vi "创建任务.vi"(0 "输入通道":tag="Dev2/ai0", 1 "最小测量范围":dbl=-500.0 format="%#_13g", 2 "最大测量范围":dbl=500.0 format="%#_13g", 9 "速率":dbl=200000.0 format="%#_13g", 11 "采样数":i32=2000, 12 "最小输入值":dbl=-2.0 format="%#_13g", 13 "最大输入值":dbl=2.0 format="%#_13g") -> (4 "task out":refnum<k21> caption="任务输出", 6 "采样数out":i32=2000, 15 "error out":errorcluster caption="错误输出")   [LabVIEW 2025]
uses:
  <resource>/objmgr/daqmx.rc
panel:
  in  "接线配置":i32(ring)=10083 items=["默认"=-1, "RSE"=10083, "NRSE"=10078, "差分"=10106, "伪差分"=12529]
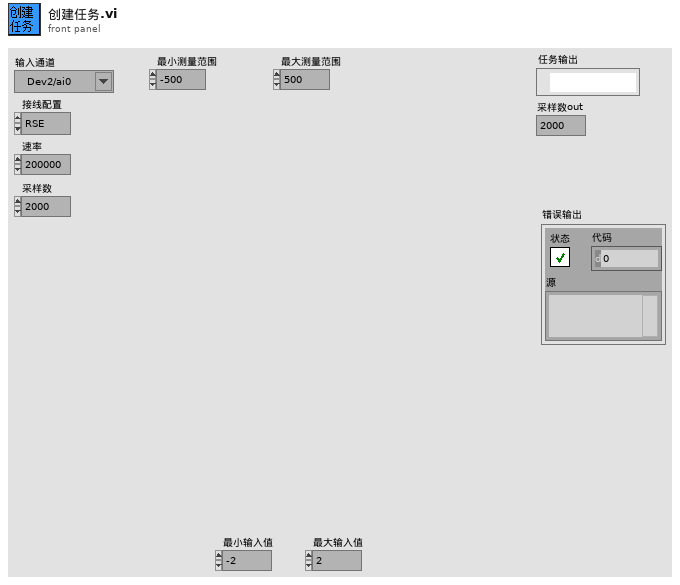
[diagram p1: front panel]
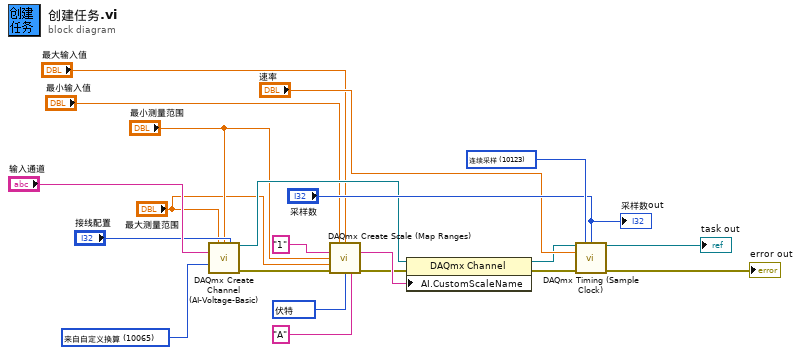
[diagram p0: block diagram]
diagram:
  w8 = 10348 items=["伏特"=10348, "A"=10342, "Deg F"=10144, "Deg C"=10143, "Deg R"=10145, "Kelvins"=10325, "应变"=10299, "欧姆"=10384, "Hz"=10373, "秒"=10364, "米"=10219, "英寸"=10379, "角度"=10146, "弧度"=10273, "时钟滴答"=10304, "g"=10186, "m/s^2"=12470, "m/s"=15959, "in/s"=15960, "帕"=10081, "Newtons"=15875, "Pounds"=15876, "kgf"=15877, "psi"=15879, "bar"=15880, "Nm"=15881, "oz-in"=15882, "lb-in"=15883, "lb-ft"=15884, "Volts/Volt"=15896, "mVolts/Volt"=15897, "来自TEDS"=12516] ("pre-scaled units")
  w15 = 10065 items=["伏特"=10348, "来自自定义换算"=10065] ("units")
  w19 = 10123 items=["有限采样"=10178, "连续采样"=10123, "硬件定时单点"=12522] ("sample mode")
  n1 = call <vilib>:"DAQmx Create Channel (AI-Voltage-Basic).vi"("maximum value"="最大测量范围", "minimum value"="最小测量范围", "input terminal configuration"="接线配置", "physical channels"="输入通道", "units"=w15) -> ("task out"=w13:refnum<k21>, "error out"=w4:errorcluster)  [unwired: 9 in]
  n2 = call <vilib>:"DAQmx Create Scale (Map Ranges).vi"("pre-scaled minimum"="最小输入值", "pre-scaled maximum"="最大输入值", "name"="1", "scaled minimum"="最小测量范围", "scaled maximum"="最大测量范围", "error in"=w4, "pre-scaled units"=w8, "scaled units"="A") -> ("scale out"=w16:tag, "error out"=w3:errorcluster)  [unwired: 6 in]
  n3 = property class="DAQmx Channel"(reference=w13, error in=w3, "AI.CustomScaleName"=w16) -> (reference out=w12:refnum<k21>, error out=w2:errorcluster)
  n4 = call <vilib>:"DAQmx Timing (Sample Clock).vi"("task/channels in"=w12, "sample mode"=w19, "samples per channel"="采样数", "rate"="速率", "error in"=w2) -> ("task out"=→"task out":refnum<k21>, "error out"=→"error out":errorcluster)  [unwired: 9 in]
  "采样数out" <- "采样数"
